vi "ZM-CP-publish.vi"(8 "error in (no error)":errorcluster, 10 "package":refnum<class "ZM-PC-package.lvclass">, 11 "ZM-CP-FL-file_logger in":refnum<class "ZM-CP-FL-file_logger.lvclass">) -> (0 "error out":errorcluster, 3 "ZM-CP-FL-file_logger out":refnum<class "ZM-CP-FL-file_logger.lvclass">)   [LabVIEW 2020, in "ZM-CP-FL-file_logger.lvlib" / "ZM-CP-FL-file_logger.lvclass"]
doc: "The file logger's ZM-CP-publish: appends the package's JSON as one line to <outputFolder>/<type>.jsonl, one file per package type. The protocol never looks inside the package. No Call Parent."
uses:
  ZM-CP-FL-file_logger.lvclass
  common/ZM-PC-packages/ZM-PC-package/ZM-PC-package.lvclass
  ZM-CP-FL-file_logger.lvclass/ZM-CP-FL-file_logger.ctl
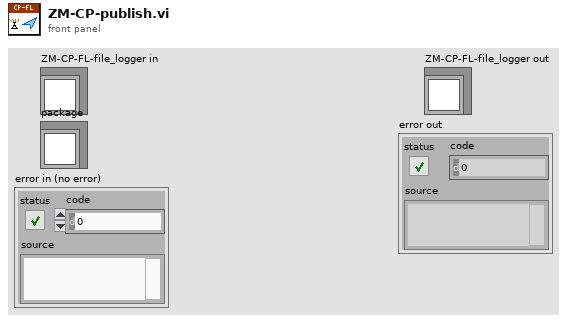
[diagram p1: front panel]
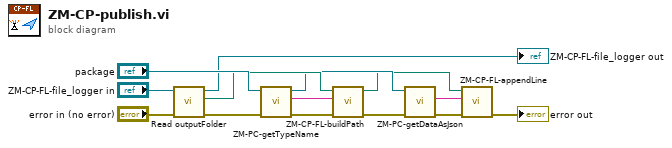
[diagram p0: block diagram]
diagram:
  n1 = call "Read outputFolder.vi"("error in (no error)"="error in (no error)", "ZM-CP-FL-file_logger in"="ZM-CP-FL-file_logger in") -> ("error out"=w11:errorcluster, "outputFolder"=w10:path, "ZM-CP-FL-file_logger out"=→"ZM-CP-FL-file_logger out":refnum<class "ZM-CP-FL-file_logger.lvclass">)  [unwired: 7 in]
  n2 = call "ZM-PC-getTypeName.vi"("error in (no error)"=w11, "ZM-PC-package in"="package") -> ("error out"=w8:errorcluster, "type_name"=w9:string, "ZM-PC-package out"=w7:refnum<class "ZM-PC-package.lvclass">)  [unwired: 7 in]
  n3 = call "ZM-CP-FL-buildPath.vi"("error in (no error)"=w8, "type_name"=w9, "folder"=w10) -> ("error out"=w6:errorcluster, "file"=w5:path)  [unwired: 7 in]
  n4 = call-dynamic "ZM-PC-getDataAsJson.vi"("error in (no error)"=w6, "ZM-PC-package in"=w7) -> ("error out"=w3:errorcluster, "json"=w4:string)  [unwired: 7 in, 1 out]
  n5 = call "ZM-CP-FL-appendLine.vi"("error in (no error)"=w3, "line"=w4, "file"=w5) -> ("error out"=→"error out":errorcluster)  [unwired: 8 in]
